vi "Copy.vi"(8 "error in":errorcluster, 9 "Target Folder":path, 10 "Source File":path, 11 "IFile Manager in":refnum<class "IFile Manager.lvclass">) -> (0 "error out":errorcluster, 2 "New Path":path, 3 "IFile Manager out":refnum<class "IFile Manager.lvclass">)   [LabVIEW 2026, in "IFile Manager.lvclass"]
doc: "This VI copies the specified source file to the target directory. If the target already exists it will be overwritten."
uses:
  IFile Manager.lvclass
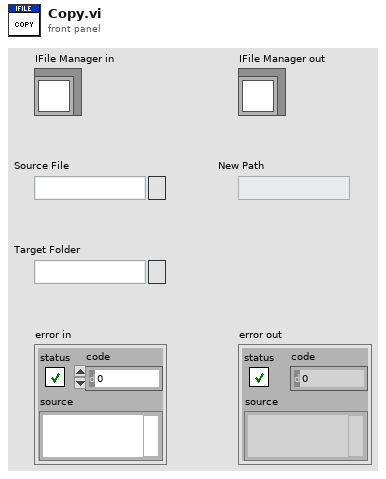
[diagram p1: front panel]
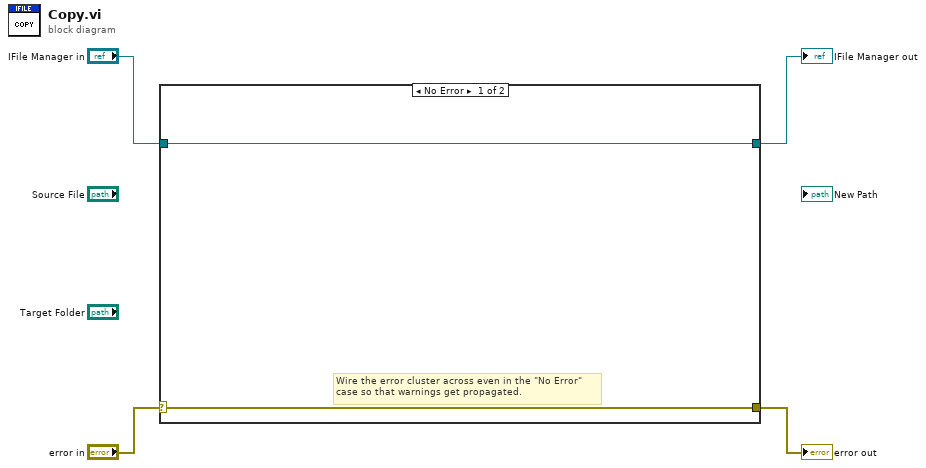
[diagram p0: block diagram]
diagram:
  n1 = case shown="No Error" "error in" {
    selector: "error in" -> [w6 w8]
    tunnel: [w6 w8] -> w3
    tunnel: [w5 w7] -> w1
    tunnel: "IFile Manager in" -> [w5 w7]
    frame No Error {
      # "Wire the error cluster across even in the \"No Error\"\ncase so that warnings get propagated."
    }
    frame Error {
    }
  }
  "error out" <- w3
  "IFile Manager out" <- w1
